vi "Variable glob Pt.vi"() -> ()   [LabVIEW 2022 SP3]
panel:
  in  "Donnees Pt/tache":cluster{"Donnees Pt":string[]}[](array[cluster])
  in  "Taches Pt 100":T1(array[cluster])
  in  "Temp Pt":bool
  out "Nb de chassis Pt":u8
  # "Platines"
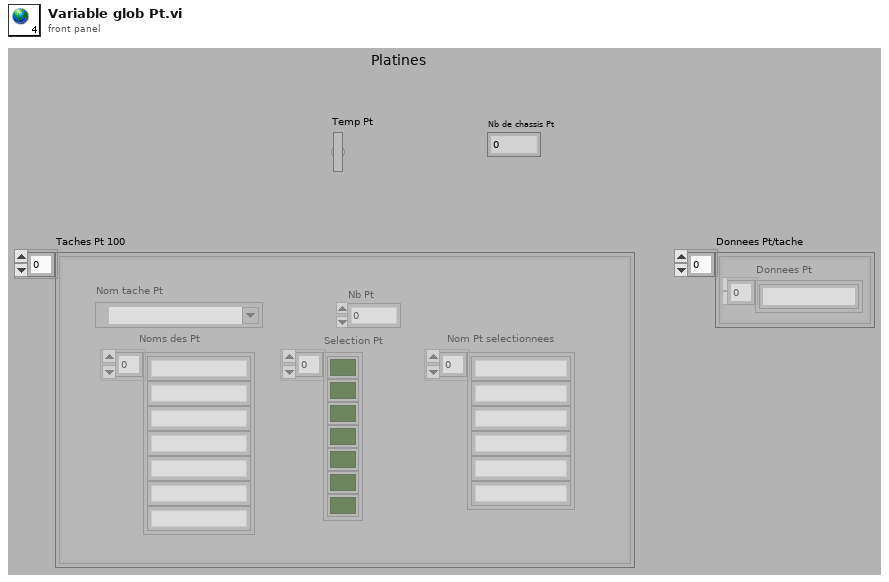
[diagram p1: front panel]
types:
  T1 = cluster{"Nom tache Pt":refnum<k21>, "Noms des Pt":string[], "Nb Pt":i16, "Selection Pt":bool[], "Nom Pt selectionnees":string[]}[]
diagram:
